vi "test request state refused.vi"(8 "error in (no error)":errorcluster) -> (0 "error out":errorcluster, 3 "body":string)   [LabVIEW 2020, in "MCP Server tests.lvlib"]
doc: "A requestState stands for state kept by the server and is bound to the request that got it. fake_tool_two_questions is called (id 71) to get a valid requestState. A retry with requestState tampered (id 711), one with the valid requestState but the tool name fake_tool_add (params.name and Mcp-Name, id 712) and one with the valid requestState but other arguments (id 713) are each refused with HTTP 400 and the JSON-RPC error -32602 with the request id. The requests are sent with the LabVIEW HTTP Client directly."
uses:
  MCP Server tests.lvlib
  <vilib>/JDP Science/JSONtext/Next JSON Value.vi
  <vilib>/JDP Science/JSONtext/String Subset.vi
  <vilib>/JDP Science/JSONtext/Parsing/Advance past next JSON Value (inlined COPY).vi
  <vilib>/JDP Science/JSONtext/Parsing/Advance past whitespace.vi
  <vilib>/JDP Science/JSONtext/Parsing/Advance past String.vi
  <vilib>/JDP Science/JSONtext/Parsing/Advance past Number.vi
  <vilib>/JDP Science/JSONtext/Parsing/Advance past Line Ending.vi
  <vilib>/JDP Science/JSONtext/Parsing/Parse Full Path or Item Name.vi
  <vilib>/JDP Science/JSONtext/Parsing/Advance past Array.vi
  <vilib>/JDP Science/JSONtext/Parsing/Advance past Object.vi
  <vilib>/JDP Science/JSONtext/support/Error Cluster From Code.vi
  <vilib>/JDP Science/JSONtext/Offset/Find Item Locations by Path.vi
  <vilib>/addons/_JKI Toolkits/Caraya/classes/Test/Test.lvclass
  <vilib>/JDP Science/JSONtext/JSONtext.lvlib
  <vilib>/addons/_JKI Toolkits/Caraya/classes/Assert/Assert.lvclass
panel:
  out "lookup error":errorcluster
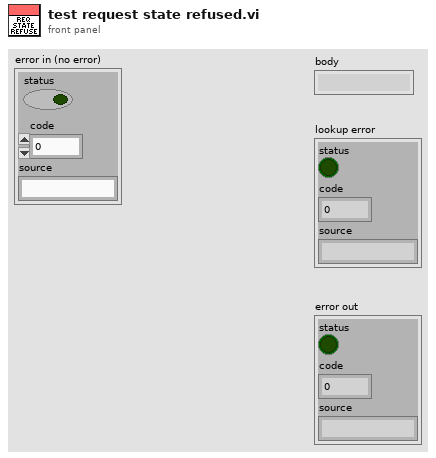
[diagram p1: front panel]
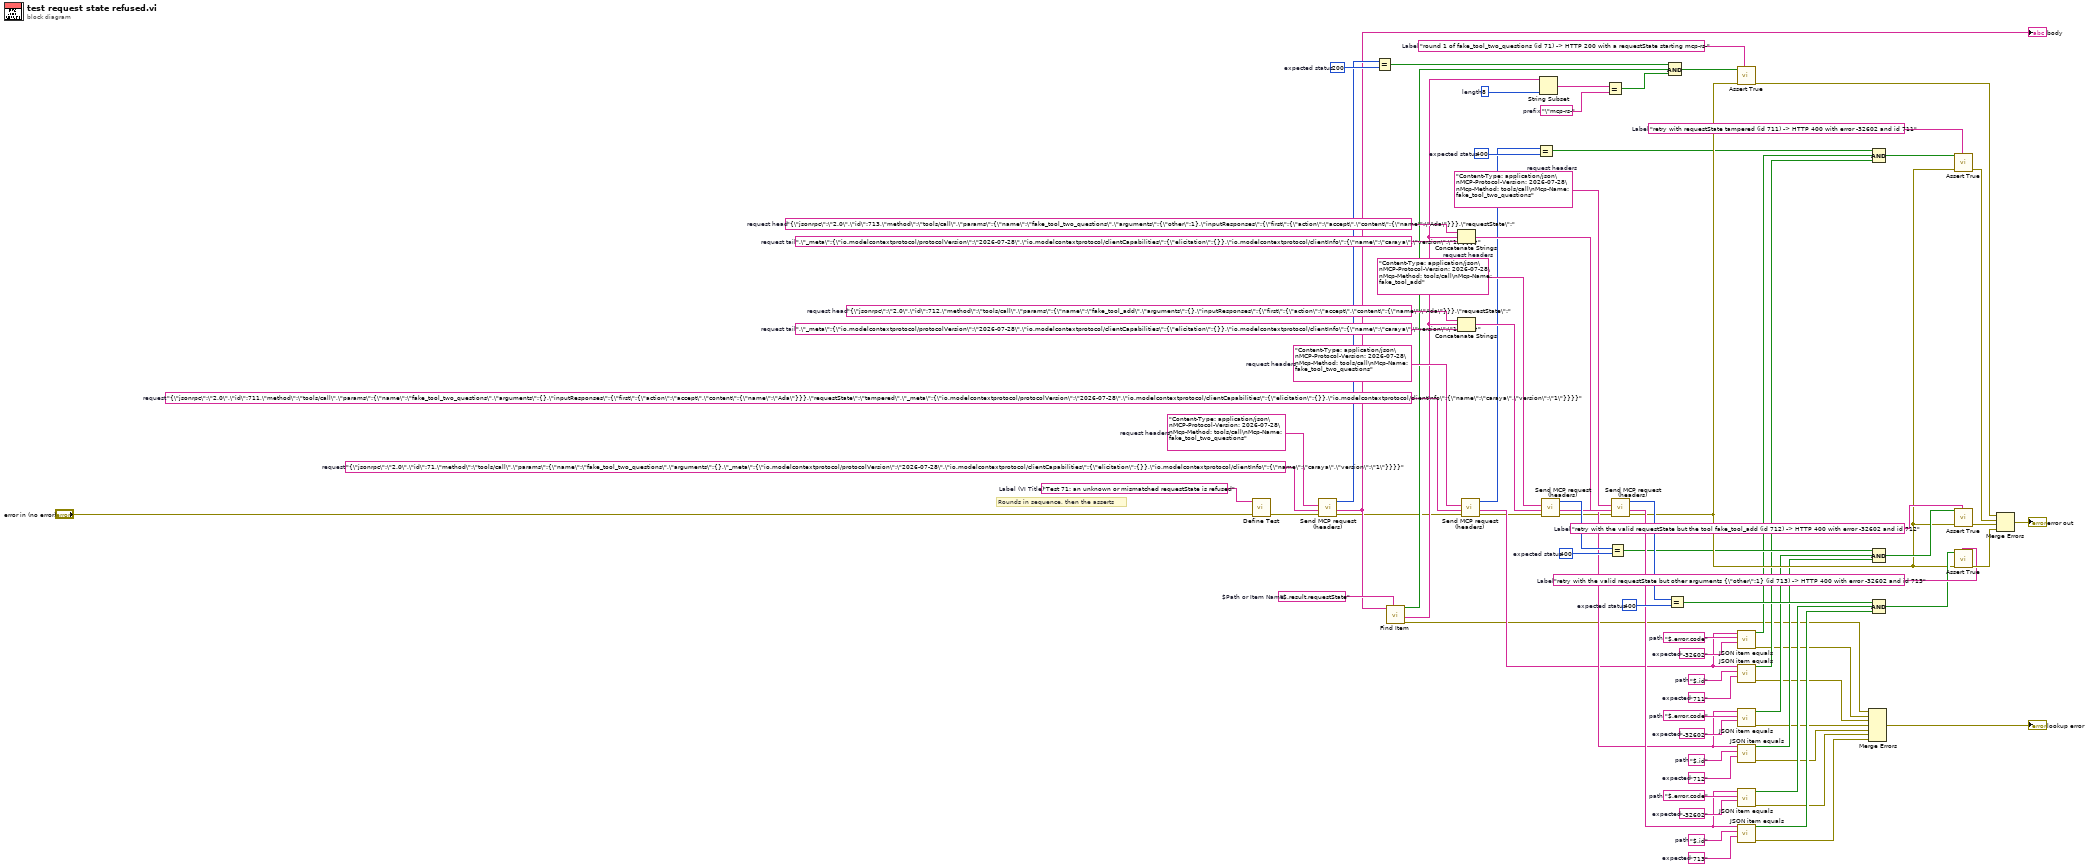
[diagram p0: block diagram]
diagram:
  w78 = "retry with the valid requestState but other arguments {\"other\":1} (id 713) -> HTTP 400 with error -32602 and id 713"  # Label
  w75 = "retry with the valid requestState but the tool fake_tool_add (id 712) -> HTTP 400 with error -32602 and id 712"  # Label
  w72 = "retry with requestState tampered (id 711) -> HTTP 400 with error -32602 and id 711"  # Label
  w69 = "round 1 of fake_tool_two_questions (id 71) -> HTTP 200 with a requestState starting mcp-rs-"  # Label
  w65 = "713"  # expected
  w64 = "$.id"  # path
  w61 = "-32602"  # expected
  w60 = "$.error.code"  # path
  w58 = 400  # expected status
  w54 = "Content-Type: application/json\nMCP-Protocol-Version: 2026-07-28\nMcp-Method: tools/call\nMcp-Name: fake_tool_two_questions"  # request headers
  w52 = ",\"_meta\":{\"io.modelcontextprotocol/protocolVersion\":\"2026-07-28\",\"io.modelcontextprotocol/clientCapabilities\":{\"elicitation\":{}},\"io.modelcontextprotocol/clientInfo\":{\"name\":\"caraya\",\"version\":\"1\"}}}}"  # request tail
  w51 = "{\"jsonrpc\":\"2.0\",\"id\":713,\"method\":\"tools/call\",\"params\":{\"name\":\"fake_tool_two_questions\",\"arguments\":{\"other\":1},\"inputResponses\":{\"first\":{\"action\":\"accept\",\"content\":{\"name\":\"Ada\"}}},\"requestState\":"  # request head
  w48 = "712"  # expected
  w47 = "$.id"  # path
  w44 = "-32602"  # expected
  w43 = "$.error.code"  # path
  w41 = 400  # expected status
  w37 = "Content-Type: application/json\nMCP-Protocol-Version: 2026-07-28\nMcp-Method: tools/call\nMcp-Name: fake_tool_add"  # request headers
  w35 = ",\"_meta\":{\"io.modelcontextprotocol/protocolVersion\":\"2026-07-28\",\"io.modelcontextprotocol/clientCapabilities\":{\"elicitation\":{}},\"io.modelcontextprotocol/clientInfo\":{\"name\":\"caraya\",\"version\":\"1\"}}}}"  # request tail
  w34 = "{\"jsonrpc\":\"2.0\",\"id\":712,\"method\":\"tools/call\",\"params\":{\"name\":\"fake_tool_add\",\"arguments\":{},\"inputResponses\":{\"first\":{\"action\":\"accept\",\"content\":{\"name\":\"Ada\"}}},\"requestState\":"  # request head
  w31 = "711"  # expected
  w30 = "$.id"  # path
  w27 = "-32602"  # expected
  w26 = "$.error.code"  # path
  w24 = 400  # expected status
  w20 = "Content-Type: application/json\nMCP-Protocol-Version: 2026-07-28\nMcp-Method: tools/call\nMcp-Name: fake_tool_two_questions"  # request headers
  w19 = "{\"jsonrpc\":\"2.0\",\"id\":711,\"method\":\"tools/call\",\"params\":{\"name\":\"fake_tool_two_questions\",\"arguments\":{},\"inputResponses\":{\"first\":{\"action\":\"accept\",\"content\":{\"name\":\"Ada\"}}},\"requestState\":\"tampered\",\"_meta\":{\"io.modelcontextprotocol/protocolVersion\":\"2026-07-28\",\"io.modelcontextprotocol/clientCapabilities\":{\"elicitation\":{}},\"io.modelcontextprotocol/clientInfo\":{\"name\":\"caraya\",\"version\":\"1\"}}}}"  # request
  w16 = 8  # length
  w15 = "\"mcp-rs-"  # prefix
  w11 = "$.result.requestState"  # $Path or Item Name
  w9 = 200  # expected status
  w5 = "Content-Type: application/json\nMCP-Protocol-Version: 2026-07-28\nMcp-Method: tools/call\nMcp-Name: fake_tool_two_questions"  # request headers
  w4 = "{\"jsonrpc\":\"2.0\",\"id\":71,\"method\":\"tools/call\",\"params\":{\"name\":\"fake_tool_two_questions\",\"arguments\":{},\"_meta\":{\"io.modelcontextprotocol/protocolVersion\":\"2026-07-28\",\"io.modelcontextprotocol/clientCapabilities\":{\"elicitation\":{}},\"io.modelcontextprotocol/clientInfo\":{\"name\":\"caraya\",\"version\":\"1\"}}}}"  # request
  w2 = "Test 71: an unknown or mismatched requestState is refused"  # Label (VI Title)
  # "Rounds in sequence, then the asserts"
  n1 = call <vilib>:"Define Test.vi"("error in (no error)"="error in (no error)", "Label (VI Title)"=w2) -> ("error out"=w3:errorcluster)  [unwired: 8 in, 1 out]
  n2 = call "Send MCP request (headers).vi"("error in (no error)"=w3, "request"=w4, "request headers"=w5) -> ("error out"=w6:errorcluster, "response"=w7:string, "status code"=w8:i32)  [unwired: 5 in, 1 out]
  "body" <- w7
  n3 = Equal?(x=w8, y=w9) -> (x = y?=w10:bool)
  n4 = call <vilib>:"Find Item.vi"("$Path or Item Name"=w11, "JSON"=w7) -> ("error out"=w12:errorcluster, "<JSON>"=w13:string, "Found"=w14:bool)  [unwired: 6 in, 1 out]
  n5 = Concatenate Strings(w51, w13, w52) -> (w53:string)
  n6 = Concatenate Strings(w34, w13, w35) -> (w36:string)
  n7 = call "Send MCP request (headers).vi"("error in (no error)"=w6, "request"=w19, "request headers"=w20) -> ("error out"=w21:errorcluster, "response"=w22:string, "status code"=w23:i32)  [unwired: 5 in, 1 out]
  n8 = Equal?(x=w23, y=w24) -> (x = y?=w25:bool)
  n9 = String Subset(string=w13, length (rest)=w16) -> (substring=w17:string)  [unwired: 1 in]
  n10 = call "Send MCP request (headers).vi"("error in (no error)"=w21, "request"=w36, "request headers"=w37) -> ("error out"=w38:errorcluster, "response"=w39:string, "status code"=w40:i32)  [unwired: 5 in, 1 out]
  n11 = Equal?(x=w17, y=w15) -> (x = y?=w18:bool)
  n12 = Equal?(x=w40, y=w41) -> (x = y?=w42:bool)
  n13 = call "Send MCP request (headers).vi"("error in (no error)"=w38, "request"=w53, "request headers"=w54) -> ("error out"=w55:errorcluster, "response"=w56:string, "status code"=w57:i32)  [unwired: 5 in, 1 out]
  n14 = Compound Arithmetic op=AND(w10, w14, w18) -> (w68:bool)
  n15 = Equal?(x=w57, y=w58) -> (x = y?=w59:bool)
  n16 = call <vilib>:"Assert True.vi"("Label"=w69, "error in (no error)"=w55, "True?"=w68) -> ("error out"=w70:errorcluster)  [unwired: 7 in, 1 out]
  n17 = call "JSON item equals.vi"("expected"=w27, "path"=w26, "JSON"=w22) -> ("error out"=w28:errorcluster, "equal?"=w29:bool)  [unwired: 6 in, 1 out]
  n18 = call "JSON item equals.vi"("expected"=w31, "path"=w30, "JSON"=w22) -> ("error out"=w32:errorcluster, "equal?"=w33:bool)  [unwired: 6 in, 1 out]
  n19 = call "JSON item equals.vi"("expected"=w44, "path"=w43, "JSON"=w39) -> ("error out"=w45:errorcluster, "equal?"=w46:bool)  [unwired: 6 in, 1 out]
  n20 = call "JSON item equals.vi"("expected"=w48, "path"=w47, "JSON"=w39) -> ("error out"=w49:errorcluster, "equal?"=w50:bool)  [unwired: 6 in, 1 out]
  n21 = call "JSON item equals.vi"("expected"=w61, "path"=w60, "JSON"=w56) -> ("error out"=w62:errorcluster, "equal?"=w63:bool)  [unwired: 6 in, 1 out]
  n22 = call "JSON item equals.vi"("expected"=w65, "path"=w64, "JSON"=w56) -> ("error out"=w66:errorcluster, "equal?"=w67:bool)  [unwired: 6 in, 1 out]
  n23 = Merge Errors(w12, w28, w32, w45, w49, w62, w66) -> (→"lookup error":errorcluster)
  n24 = Compound Arithmetic op=AND(w25, w29, w33) -> (w71:bool)
  n25 = Compound Arithmetic op=AND(w42, w46, w50) -> (w74:bool)
  n26 = Compound Arithmetic op=AND(w59, w63, w67) -> (w77:bool)
  n27 = call <vilib>:"Assert True.vi"("Label"=w72, "error in (no error)"=w55, "True?"=w71) -> ("error out"=w73:errorcluster)  [unwired: 7 in, 1 out]
  n28 = call <vilib>:"Assert True.vi"("Label"=w75, "error in (no error)"=w55, "True?"=w74) -> ("error out"=w76:errorcluster)  [unwired: 7 in, 1 out]
  n29 = call <vilib>:"Assert True.vi"("Label"=w78, "error in (no error)"=w55, "True?"=w77) -> ("error out"=w79:errorcluster)  [unwired: 7 in, 1 out]
  n30 = Merge Errors(w70, w73, w76, w79) -> (→"error out":errorcluster)
